vi "Configure Module.vi"(8 "error in (no error)":errorcluster, 10 "IOV ref in":variant, 11 "Module Template in":refnum<class "9205.lvclass">) -> (0 "error out":errorcluster, 2 "IOV ref out":variant, 3 "Module Template out":refnum<class "9205.lvclass">)   [LabVIEW 2020, in "Modules.lvlib" / "9205.lvclass"]
uses:
  9205.lvclass
  <resource>/objmgr/cRIO.rc
  RSI Module/RSI Module.lvclass
  C:/Users/nitest/Desktop/Git 2020/niveristand-scan-engine-module-libraries/Source/RSI Module/RSI Module.lvclass
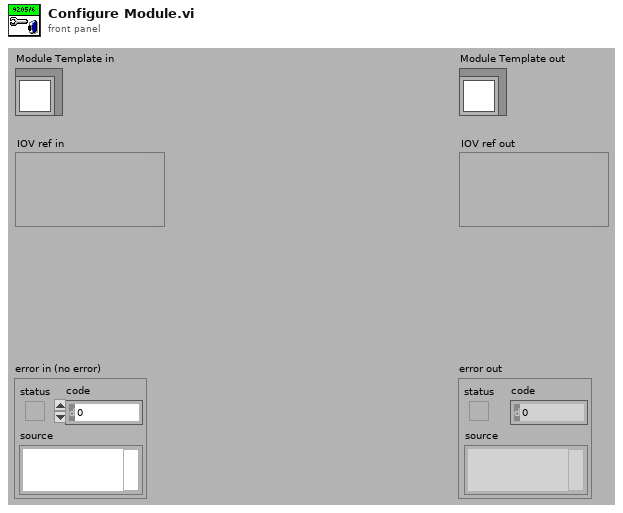
[diagram p1: front panel]
types:
  T1 = typedef "Modules.lvlib/9205.lvclass/Channel Settings.ctl" = cluster{"Range":T2, "Terminal mode":T3}[]
  T2 = typedef "Modules.lvlib/9205.lvclass/Range.ctl" = u32
  T3 = typedef "Modules.lvlib/9205.lvclass/Terminal mode.ctl" = u32
  T4 = typedef "Modules.lvlib/RSI Module.lvclass/Module Models.ctl" = enum16{"Empty", "NI 9201", "NI 9203", "NI 9205", "NI 9206", "NI 9207", "NI 9208", "NI 9209", "NI 9210", "NI 9211", "NI 9212", "NI 9213", "NI 9214", "NI 9215", "NI 9216", "NI 9217", "NI 9219", "NI 9220", "NI 9221", "NI 9222", "NI 9223", "NI 9224", "NI 9225", "NI 9226", "NI 9227", "NI 9228", "NI 9229", "NI 9233", "NI 9234", "NI 9235", "NI 9236", "NI 9237", "NI 9239", "NI 9242", "NI 9244", "NI 9253", "NI 9263", "NI 9264", "NI 9265", "NI 9266", "NI 9269", "NI 9344", "NI 9350", "NI 9375", "NI 9401", "NI 9402", "NI 9403", "NI 9411", "NI 9421", "NI 9422", "NI 9423", "NI 9425", "NI 9426", "NI 9435", "NI 9436", "NI 9437", "NI 9472", "NI 9474", "NI 9475", "NI 9476", "NI 9477", "NI 9478", "NI 9481", "NI 9482", "NI 9485"}
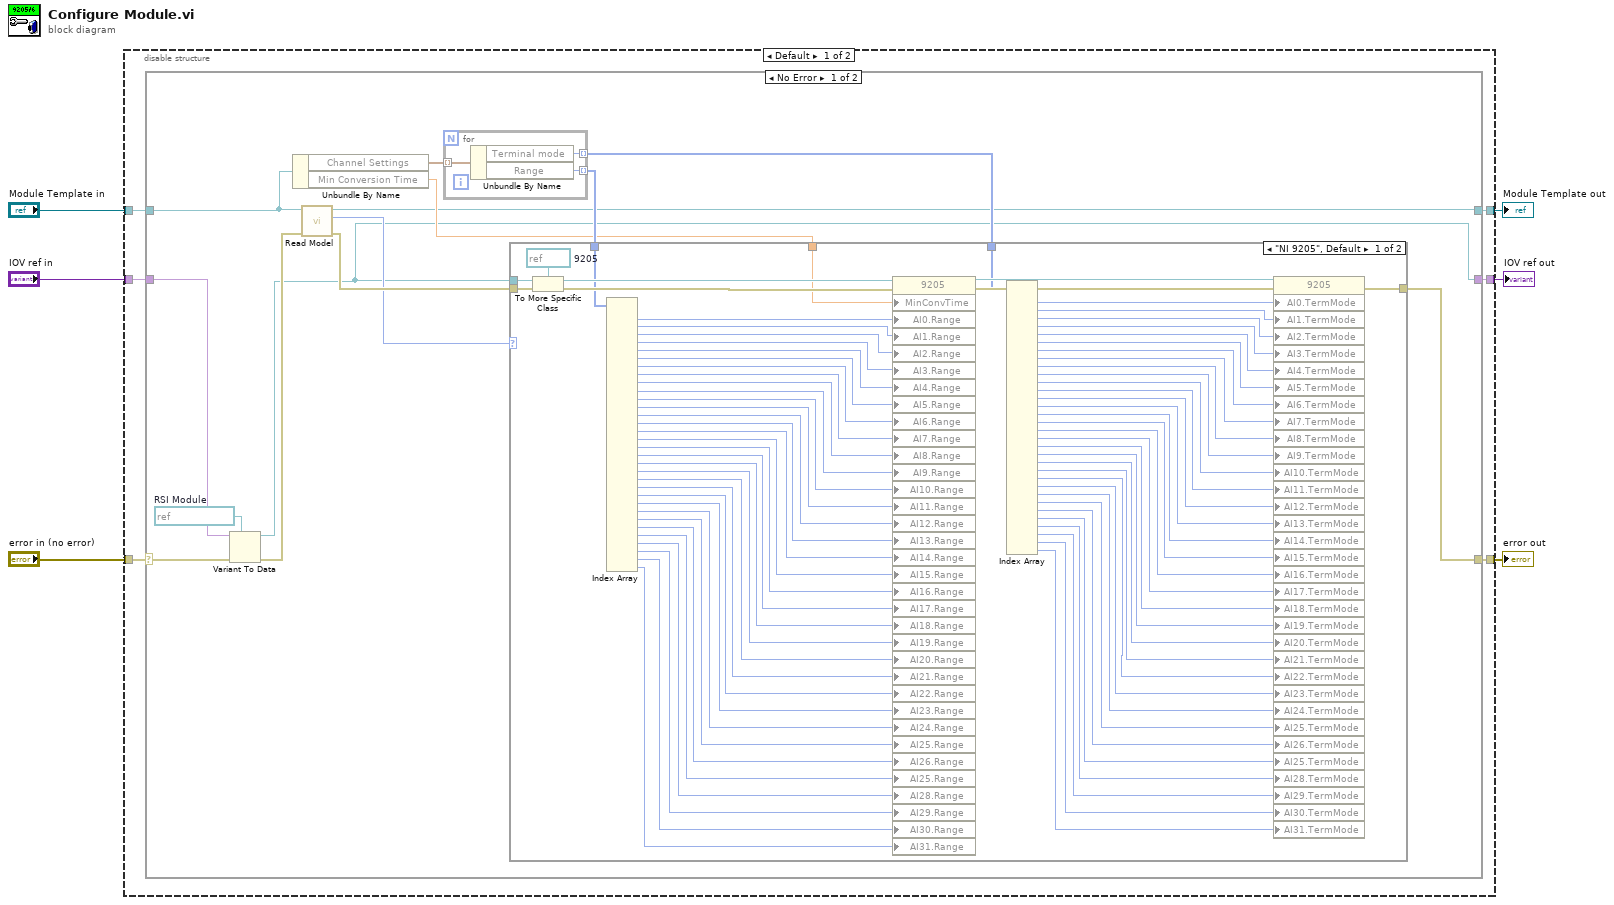
[diagram p0: block diagram]
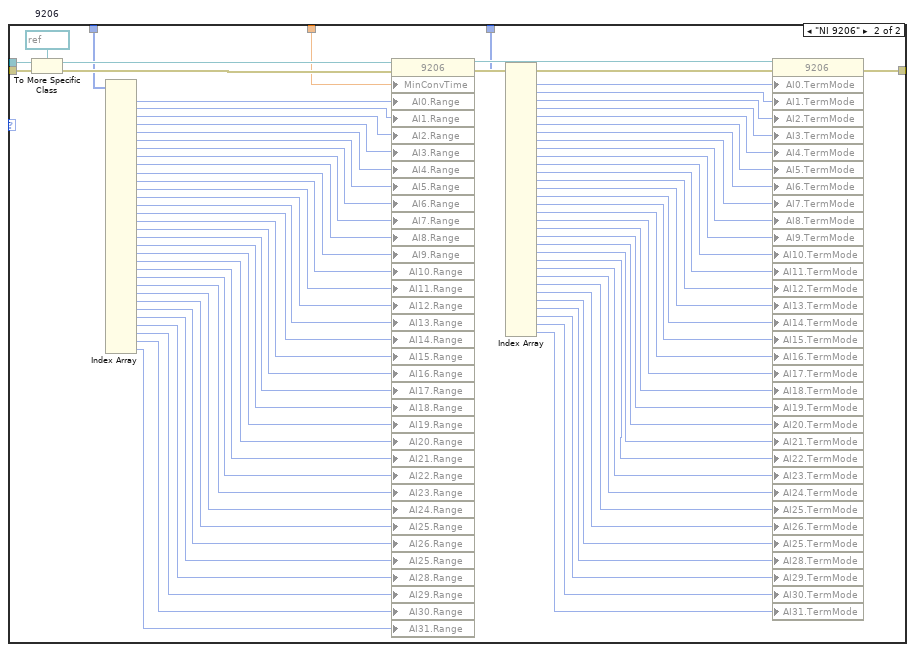
[diagram p2: hidden frame]
diagram:
  n1 = disable-structure shown="Default" {
    disable-tunnel: "error in (no error)" -> [w12 w185]
    disable-tunnel: [w11 w185] -> w5
    disable-tunnel: "Module Template in" -> [w10 w183]
    disable-tunnel: [w9 w183] -> w3
    disable-tunnel: "IOV ref in" -> [w8 w184]
    disable-tunnel: [w7 w184] -> w1
    frame condition #0 {
      n2 = case shown="No Error" w12 {
        selector: w12 -> [w19 w182]
        tunnel: [w25 w182] -> w11
        tunnel: [w20 w181] -> w9
        tunnel: w10 -> [w21 w181]
        tunnel: w8 -> [w15 w180]
        tunnel: [w14 w180] -> w7
        frame No Error {
          w13 = refnum<k21> refnum  # RSI Module
          n3 = Variant To Data(error in=w19, type=w13, Variant=w15) -> (data=w14:refnum<k21>, error out=w16:errorcluster)
          n4 = Unbundle By Name(w21) -> ("Channel Settings"=w26:T1, "Min Conversion Time"=w22:dbl)
          n5 = call "Read Model.vi"("error in (no error)"=w16, "RSI Module in"=w21) -> ("error out"=w18:errorcluster, "Model"=w17:T4, "RSI Module out"=w20:refnum<class "9205.lvclass">)  [unwired: 7 in]
          n6 = for {
            tunnel: w26 -> [w179] mode=indexing
            tunnel: [w178] -> w23 mode=indexing
            tunnel: [w177] -> w24 mode=indexing
            n7 = Unbundle By Name(w179) -> ("Terminal mode"=w178:T3, "Range"=w177:T2)
          }
          n8 = case shown="\"NI 9205\", Default" w17 {
            tunnel: w18 -> [w101 w176]
            tunnel: w14 -> [w97 w172]
            tunnel: [w94 w169] -> w25
            tunnel: w24 -> [w93 w168]
            tunnel: w23 -> [w61 w136]
            tunnel: w22 -> [w59 w134]
            frame "NI 9205", Default {
              w100 = refnum<k21> refnum  # 9205
              n9 = To More Specific Class(target class=w100, reference=w97, error in=w101) -> (specific class reference=w99:refnum<k21>, error out=w98:errorcluster)
              n10 = Index Array(array=w93) -> (element #1=w60:T2, element #2=w92:T2, element #3=w91:T2, element #4=w90:T2, element #5=w89:T2, element #6=w88:T2, element #7=w87:T2, element #8=w86:T2, element #9=w85:T2, element #10=w84:T2, element #11=w83:T2, element #12=w82:T2, element #13=w81:T2, element #14=w80:T2, element #15=w79:T2, element #16=w78:T2, element #17=w77:T2, element #18=w76:T2, element #19=w75:T2, element #20=w74:T2, element #21=w73:T2, element #22=w72:T2, element #23=w71:T2, element #24=w70:T2, element #25=w69:T2, element #26=w68:T2, element #27=w67:T2, element #28=w66:T2, element #29=w65:T2, element #30=w64:T2, element #31=w63:T2, element #32=w62:T2)  [unwired: 32 in]
              n11 = property class="9205"(reference=w99, error in=w98, "MinConvTime"=w59, "AI0.Range"=w60, "AI1.Range"=w92, "AI2.Range"=w91, "AI3.Range"=w90, "AI4.Range"=w89, "AI5.Range"=w88, "AI6.Range"=w87, "AI7.Range"=w86, "AI8.Range"=w85, "AI9.Range"=w84, "AI10.Range"=w83, "AI11.Range"=w82, "AI12.Range"=w81, "AI13.Range"=w80, "AI14.Range"=w79, "AI15.Range"=w78, "AI16.Range"=w77, "AI17.Range"=w76, "AI18.Range"=w75, "AI19.Range"=w74, "AI20.Range"=w73, "AI21.Range"=w72, "AI22.Range"=w71, "AI23.Range"=w70, "AI24.Range"=w69, "AI25.Range"=w68, "AI26.Range"=w67, "AI25.Range"=w66, "AI28.Range"=w65, "AI29.Range"=w64, "AI30.Range"=w63, "AI31.Range"=w62) -> (reference out=w96:refnum<k21>, error out=w95:errorcluster)
              n12 = Index Array(array=w61) -> (element #1=w58:T3, element #2=w57:T3, element #3=w56:T3, element #4=w55:T3, element #5=w54:T3, element #6=w53:T3, element #7=w52:T3, element #8=w51:T3, element #9=w50:T3, element #10=w49:T3, element #11=w48:T3, element #12=w47:T3, element #13=w46:T3, element #14=w45:T3, element #15=w44:T3, element #16=w43:T3, element #17=w42:T3, element #18=w41:T3, element #19=w40:T3, element #20=w39:T3, element #21=w38:T3, element #22=w37:T3, element #23=w36:T3, element #24=w35:T3, element #25=w34:T3, element #26=w33:T3, element #27=w32:T3, element #28=w31:T3, element #29=w30:T3, element #30=w29:T3, element #31=w28:T3, element #32=w27:T3)  [unwired: 32 in]
              n13 = property class="9205"(reference=w96, error in=w95, "AI0.TermMode"=w58, "AI1.TermMode"=w57, "AI2.TermMode"=w56, "AI3.TermMode"=w55, "AI4.TermMode"=w54, "AI5.TermMode"=w53, "AI6.TermMode"=w52, "AI7.TermMode"=w51, "AI8.TermMode"=w50, "AI9.TermMode"=w49, "AI10.TermMode"=w48, "AI11.TermMode"=w47, "AI12.TermMode"=w46, "AI13.TermMode"=w45, "AI14.TermMode"=w44, "AI15.TermMode"=w43, "AI16.TermMode"=w42, "AI17.TermMode"=w41, "AI18.TermMode"=w40, "AI19.TermMode"=w39, "AI20.TermMode"=w38, "AI21.TermMode"=w37, "AI22.TermMode"=w36, "AI23.TermMode"=w35, "AI24.TermMode"=w34, "AI25.TermMode"=w33, "AI26.TermMode"=w32, "AI25.TermMode"=w31, "AI28.TermMode"=w30, "AI29.TermMode"=w29, "AI30.TermMode"=w28, "AI31.TermMode"=w27) -> (error out=w94:errorcluster)  [unwired: 1 out]
            }
            frame "NI 9206" {
              w175 = refnum<k21> refnum  # 9206
              n14 = To More Specific Class(target class=w175, reference=w172, error in=w176) -> (specific class reference=w174:refnum<k21>, error out=w173:errorcluster)
              n15 = Index Array(array=w168) -> (element #1=w135:T2, element #2=w167:T2, element #3=w166:T2, element #4=w165:T2, element #5=w164:T2, element #6=w163:T2, element #7=w162:T2, element #8=w161:T2, element #9=w160:T2, element #10=w159:T2, element #11=w158:T2, element #12=w157:T2, element #13=w156:T2, element #14=w155:T2, element #15=w154:T2, element #16=w153:T2, element #17=w152:T2, element #18=w151:T2, element #19=w150:T2, element #20=w149:T2, element #21=w148:T2, element #22=w147:T2, element #23=w146:T2, element #24=w145:T2, element #25=w144:T2, element #26=w143:T2, element #27=w142:T2, element #28=w141:T2, element #29=w140:T2, element #30=w139:T2, element #31=w138:T2, element #32=w137:T2)  [unwired: 32 in]
              n16 = property class="9206"(reference=w174, error in=w173, "MinConvTime"=w134, "AI0.Range"=w135, "AI1.Range"=w167, "AI2.Range"=w166, "AI3.Range"=w165, "AI4.Range"=w164, "AI5.Range"=w163, "AI6.Range"=w162, "AI7.Range"=w161, "AI8.Range"=w160, "AI9.Range"=w159, "AI10.Range"=w158, "AI11.Range"=w157, "AI12.Range"=w156, "AI13.Range"=w155, "AI14.Range"=w154, "AI15.Range"=w153, "AI16.Range"=w152, "AI17.Range"=w151, "AI18.Range"=w150, "AI19.Range"=w149, "AI20.Range"=w148, "AI21.Range"=w147, "AI22.Range"=w146, "AI23.Range"=w145, "AI24.Range"=w144, "AI25.Range"=w143, "AI26.Range"=w142, "AI25.Range"=w141, "AI28.Range"=w140, "AI29.Range"=w139, "AI30.Range"=w138, "AI31.Range"=w137) -> (reference out=w171:refnum<k21>, error out=w170:errorcluster)
              n17 = Index Array(array=w136) -> (element #1=w133:T3, element #2=w132:T3, element #3=w131:T3, element #4=w130:T3, element #5=w129:T3, element #6=w128:T3, element #7=w127:T3, element #8=w126:T3, element #9=w125:T3, element #10=w124:T3, element #11=w123:T3, element #12=w122:T3, element #13=w121:T3, element #14=w120:T3, element #15=w119:T3, element #16=w118:T3, element #17=w117:T3, element #18=w116:T3, element #19=w115:T3, element #20=w114:T3, element #21=w113:T3, element #22=w112:T3, element #23=w111:T3, element #24=w110:T3, element #25=w109:T3, element #26=w108:T3, element #27=w107:T3, element #28=w106:T3, element #29=w105:T3, element #30=w104:T3, element #31=w103:T3, element #32=w102:T3)  [unwired: 32 in]
              n18 = property class="9206"(reference=w171, error in=w170, "AI0.TermMode"=w133, "AI1.TermMode"=w132, "AI2.TermMode"=w131, "AI3.TermMode"=w130, "AI4.TermMode"=w129, "AI5.TermMode"=w128, "AI6.TermMode"=w127, "AI7.TermMode"=w126, "AI8.TermMode"=w125, "AI9.TermMode"=w124, "AI10.TermMode"=w123, "AI11.TermMode"=w122, "AI12.TermMode"=w121, "AI13.TermMode"=w120, "AI14.TermMode"=w119, "AI15.TermMode"=w118, "AI16.TermMode"=w117, "AI17.TermMode"=w116, "AI18.TermMode"=w115, "AI19.TermMode"=w114, "AI20.TermMode"=w113, "AI21.TermMode"=w112, "AI22.TermMode"=w111, "AI23.TermMode"=w110, "AI24.TermMode"=w109, "AI25.TermMode"=w108, "AI26.TermMode"=w107, "AI25.TermMode"=w106, "AI28.TermMode"=w105, "AI29.TermMode"=w104, "AI30.TermMode"=w103, "AI31.TermMode"=w102) -> (error out=w169:errorcluster)  [unwired: 1 out]
            }
          }
        }
        frame Error {
        }
      }
    }
    frame condition #1 (active) {
    }
  }
  "error out" <- w5
  "Module Template out" <- w3
  "IOV ref out" <- w1
